vi "TxCommit_Core.vi"(8 "error in (no error)":errorcluster, 11 "DBC in":refnum<class "DBC.lvclass">) -> (0 "error out":errorcluster, 3 "DBC out":refnum<class "DBC.lvclass">)   [LabVIEW 2020, in "ORM_pgsql_jdp.lvlib" / "DBC.lvclass"]
uses:
  DBC.lvclass
  DBC.lvclass/DBC.ctl
  <vilib>/JDP Science/PostgreSQL Library/Connection/Execute (no results).vi
  <vilib>/JDP Science/PostgreSQL Library/Connection/Execute (Return first result with rows).vi
  <vilib>/JDP Science/PostgreSQL Library/Connection/Execute Single Statement (String Parameters).vi
  <vilib>/JDP Science/PostgreSQL Library/Result/Clear.vi
  <vilib>/JDP Science/PostgreSQL Library/Connection/PQ Connection.lvclass
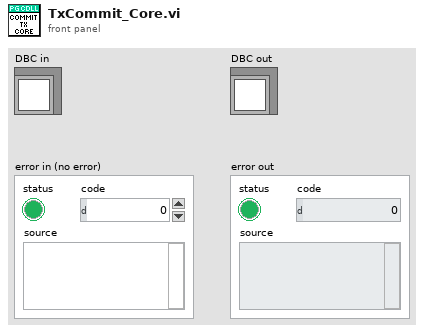
[diagram p1: front panel]
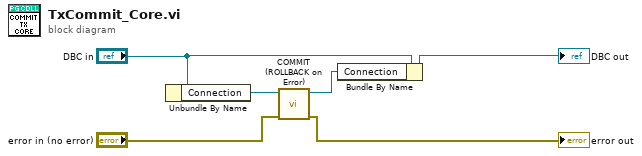
[diagram p0: block diagram]
diagram:
  n1 = Unbundle By Name("DBC in") -> ("Connection"=w5:refnum<class "PQ Connection.lvclass">)
  n2 = call <vilib>:"COMMIT (ROLLBACK on Error).vi"("error in (no error)"="error in (no error)", "PQ Connection in"=w5) -> ("error out"=→"error out":errorcluster, "PQ Connection out"=w1:refnum<class "PQ Connection.lvclass">)  [unwired: 8 in]
  n3 = Bundle By Name(cluster="DBC in", "Connection"=w1) -> (→"DBC out":refnum<class "DBC.lvclass">)
